vi "to_json.vi"(8 "error in":errorcluster, 11 "properties in":refnum<class "properties.lvclass">) -> (0 "error out":errorcluster, 2 "json":string, 3 "properties out":refnum<class "properties.lvclass">, 4 "Not Default":bool)   [LabVIEW 2020, in "nominal types.lvlib" / "properties.lvclass"]
uses:
  properties.lvclass
  properties.lvclass/properties.ctl
  903269e2-f1d6-4134-a799-7d6a349d4ca4.vi
  <vilib>/JDP Science/JSONtext/JSONtext.lvlib
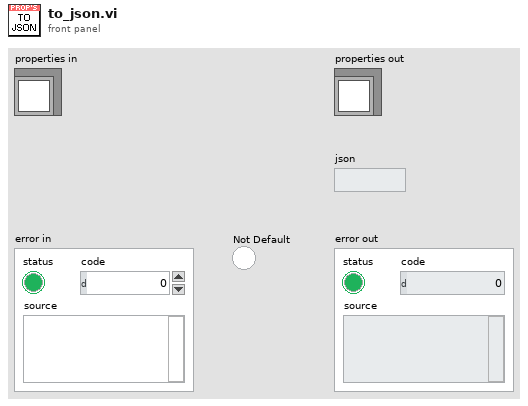
[diagram p1: front panel]
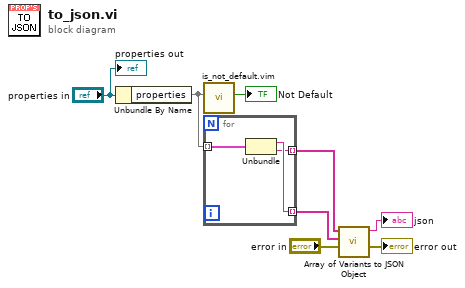
[diagram p0: block diagram]
diagram:
  n1 = Unbundle By Name("properties in") -> ("properties"=w2:map{string, string})
  n2 = call "is_not_default.vim"("data"=w2) -> ("Not Default"=→"Not Default":bool)  [unwired: 10 in]
  n3 = for {
    tunnel: w2 -> [w11] mode=indexing
    tunnel: [w10] -> w6 mode=indexing
    tunnel: [w9] -> w7 mode=indexing
    n4 = Unbundle(w11) -> ("name"=w10:string, "value"=w9:string)
  }
  n5 = call <vilib>:"Array of Variants to JSON Object.vi"("error in (no error)"="error in", "Names"=w6, "Array"=w7) -> ("error out"=→"error out":errorcluster, "<JSON>"=→"json":string)  [unwired: 7 in]
  "properties out" <- "properties in"
